vi "Write events.vi"(8 "error in (no error)":errorcluster, 10 "ZM-ROOT-EVENTS":T1, 11 "ZM-ROOT-root in":refnum<class "ZM-ROOT-root.lvclass">) -> (0 "error out":errorcluster, 3 "ZM-ROOT-root out":refnum<class "ZM-ROOT-root.lvclass">)   [LabVIEW 2020, in "ZM-ROOT-root.lvlib" / "ZM-ROOT-root.lvclass"]
doc: "Writes one field of this class's private data. Generated by lvai_create_accessors from the class private data control."
uses:
  ZM-ROOT-root.lvclass
  ZM-ROOT-root.lvclass/ZM-ROOT-root.ctl
  ZM-ROOT-EVENTS.ctl
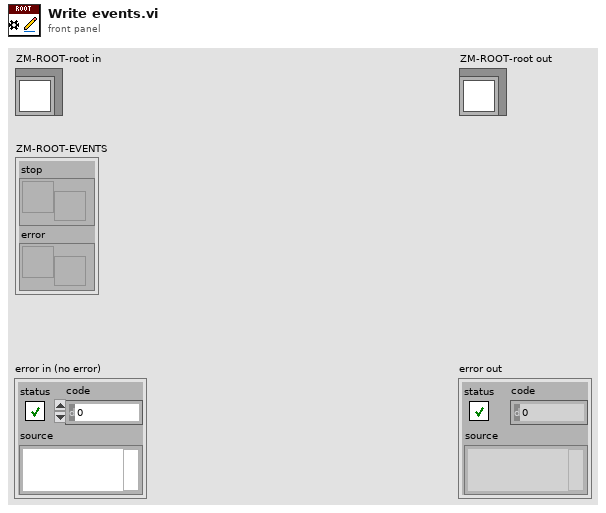
[diagram p1: front panel]
types:
  T1 = typedef "ZM-ROOT-root.lvlib/ZM-ROOT-root.lvclass/ZM-ROOT-EVENTS.ctl" = cluster{"stop":refnum<user-event>, "error":refnum<user-event>}
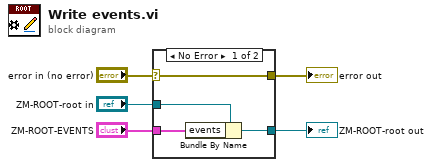
[diagram p0: block diagram]
diagram:
  n1 = case shown="No Error" "error in (no error)" {
    selector: "error in (no error)" -> [w9 w10]
    tunnel: [w9 w10] -> w4
    tunnel: [w7 w11] -> w2
    tunnel: "ZM-ROOT-root in" -> [w8 w11]
    tunnel: "ZM-ROOT-EVENTS" -> [w6 _]
    frame No Error {
      n2 = Bundle By Name(cluster=w8, "events"=w6) -> (w7:refnum<class "ZM-ROOT-root.lvclass">)
    }
    frame Error {
    }
  }
  "error out" <- w4
  "ZM-ROOT-root out" <- w2
